vi "OpenURI - Basic Example.vi"() -> ()   [LabVIEW 2013]
uses:
  uri/URI.lvclass/URI.ctl
  components/path/URI-Component.Path.lvclass/URI-Component.Path.ctl
  components/path/URI-Component.Path.lvclass
  uri/Write scheme.vi
  uri/Write port.vi
  uri/Write host.vi
  uri/Read path.vi
  uri/Read path segments.vi
  components/path/Get Segments.vi
  uri/checkCached.vi
  components/path/Get path (absolute).vi
  uri/URI.lvclass
panel:
  out "context":string
  out "port":u16
  out "Raw Segments":string[](array[string])
  out "Encoded Segments":string[](array[string])
  out "Raw Path":string
  out "Encoded Path":string
  out "set path with restricted characters":string
  out "set path by segments":string
  out "query from attributes":string
  out "changed scheme and port":string
  out "multiple query parameters":string
  out "query":string
  out "index.php":string
  out "Localhost URI":string
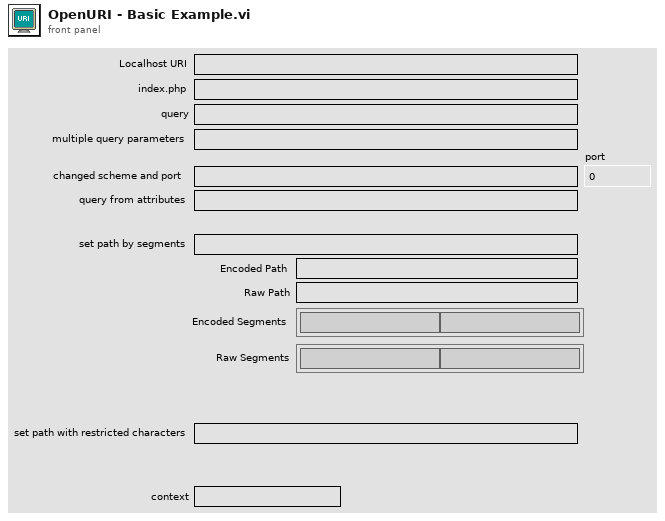
[diagram p1: front panel]
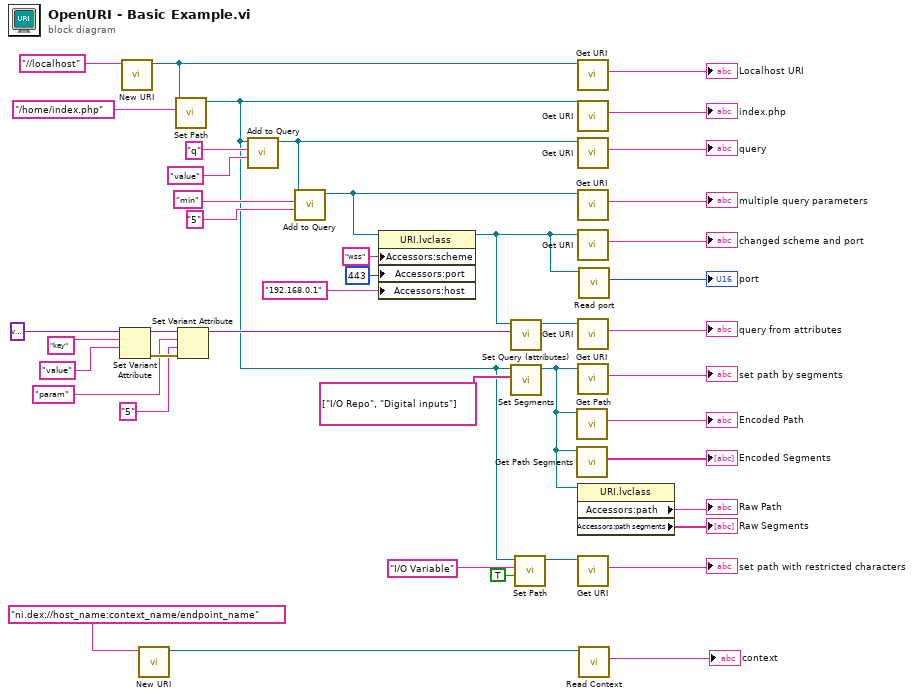
[diagram p0: block diagram]
diagram:
  n1 = Set Variant Attribute(Variant=variant ("variant"), name="key" ("path"), value="value" ("path")) -> (Variant out=w22:variant, error out=w23:errorcluster)  [unwired: 1 in, 1 out]
  n2 = call "New URI.vi"("URI"="//localhost") -> ("URI"=w42:refnum<class "URI.lvclass">)  [unwired: 9 in, 1 out]
  n3 = call "New URI.vi"("URI"="ni.dex://host_name:context_name/endpoint_name") -> ("URI"=w2:refnum<class "URI.lvclass">)  [unwired: 9 in, 1 out]
  n4 = call "Set Path.vi"("path"="/home/index.php", "URI in"=w42) -> ("URI out"=w10:refnum<class "URI.lvclass">)  [unwired: 8 in, 1 out]
  n5 = Set Variant Attribute(Variant=w22, name="param" ("path"), value="5" ("path"), error in=w23) -> (Variant out=w19:variant)  [unwired: 2 out]
  n6 = call "Add to Query.vi"("value"="value" ("path"), "key"="q" ("path"), "URI in"=w10) -> ("URI out"=w36:refnum<class "URI.lvclass">)  [unwired: 7 in, 1 out]
  n7 = call "Add to Query.vi"("value"="5" ("path"), "key"="min" ("path"), "URI in"=w36) -> ("URI out"=w32:refnum<class "URI.lvclass">)  [unwired: 7 in, 1 out]
  n8 = property class="URI.lvclass"(reference=w32, "Accessors:scheme"="wss" ("scheme"), "Accessors:port"=u16 443 ("port"), "Accessors:host"="192.168.0.1" ("scheme")) -> (reference out=w6:refnum<class "URI.lvclass">)  [unwired: 1 in, 1 out]
  n9 = call "Set Query (attributes).vi"("Query"=w19, "URI in"=w6) -> ("URI out"=w27:refnum<class "URI.lvclass">)  [unwired: 8 in, 1 out]
  n10 = call "Set Segments.vi"("Segments"=string[] ["I/O Repo", "Digital inputs"], "URI in"=w10) -> ("URI out"=w9:refnum<class "URI.lvclass">)  [unwired: 8 in, 1 out]
  n11 = call "Set Path.vi"("Encode?"=TRUE, "path"="I/O Variable", "URI in"=w10) -> ("URI out"=w14:refnum<class "URI.lvclass">)  [unwired: 7 in, 1 out]
  n12 = call "Get Path.vi"("URI in"=w9) -> ("path"=→"Encoded Path":string)  [unwired: 8 in, 2 out]
  n13 = call "Get Path Segments.vi"("URI in"=w9) -> ("Segments"=→"Encoded Segments":string[])  [unwired: 8 in, 2 out]
  n14 = call "Get URI.vi"("URI in"=w42) -> ("URI String"=→"Localhost URI":string)  [unwired: 8 in, 2 out]
  n15 = call "Get URI.vi"("URI in"=w10) -> ("URI String"=→"index.php":string)  [unwired: 8 in, 2 out]
  n16 = call "Get URI.vi"("URI in"=w36) -> ("URI String"=→"query":string)  [unwired: 8 in, 2 out]
  n17 = call "Get URI.vi"("URI in"=w32) -> ("URI String"=→"multiple query parameters":string)  [unwired: 8 in, 2 out]
  n18 = call "Get URI.vi"("URI in"=w6) -> ("URI String"=→"changed scheme and port":string)  [unwired: 8 in, 2 out]
  n19 = call "Get URI.vi"("URI in"=w27) -> ("URI String"=→"query from attributes":string)  [unwired: 8 in, 2 out]
  n20 = call "Get URI.vi"("URI in"=w9) -> ("URI String"=→"set path by segments":string)  [unwired: 8 in, 2 out]
  n21 = property class="URI.lvclass"(reference=w9) -> ("Accessors:path"=→"Raw Path":string, "Accessors:path segments"=→"Raw Segments":string[])  [unwired: 1 in, 2 out]
  n22 = call "Get URI.vi"("URI in"=w14) -> ("URI String"=→"set path with restricted characters":string)  [unwired: 8 in, 2 out]
  n23 = call "Read port.vi"("URI in"=w6) -> ("port"=→"port":u16)  [unwired: 8 in, 2 out]
  n24 = call "Read Context.vi"("URI in"=w2) -> ("context"=→"context":string)  [unwired: 8 in, 2 out]
